vi "lvmcp_propitems.vi"() -> ()   [LabVIEW 2026]
panel:
  out "Property Items[]":refnum<vi>[](array[refnum])
  out "error out":errorcluster
  in  "reference":refnum<vi>
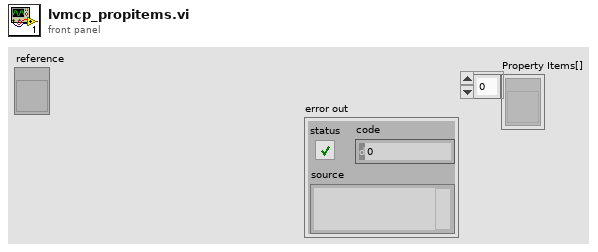
[diagram p1: front panel]
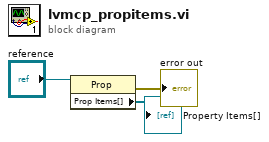
[diagram p0: block diagram]
diagram:
  n1 = property class="Prop"(reference="reference") -> (error out=→"error out":errorcluster, "Prop Items[]"=→"Property Items[]":refnum<vi>[])  [unwired: 1 in, 1 out]
